vi "UI.vi"(8 "error in (no error)":errorcluster, 11 "Node Ptr":T1 format="%.0x") -> (0 "error out":errorcluster)   [LabVIEW 2020, in "Modules.lvlib" / "9210.lvclass"]
uses:
  9210.lvclass
  <vilib>/NI VeriStand/Custom Device API/Custom Device Item Ref.ctl
  RSI Module/SubPanel Command.ctl
  C:/Users/nitest/Desktop/Git 2020/niveristand-scan-engine-module-libraries/Source/RSI Module/RSI Module.lvclass
  9210.lvclass/9210.ctl
  RSI Module/RSI Module.lvclass
  <vilib>/NI VeriStand/Custom Device API/Custom Device API.lvlib
panel:
  in  "Units":u8(ring) caption="Measurement Units" items=["Raw Volts", "Degrees Kelvin", "Degrees Celsius", "Degrees Fahrenheit", "Degrees Rankine"]
  in  "Type":u8(ring) caption="Thermocouple Type" items=["J", "K", "T", "E", "R", "S", "N", "B"]
  in  "Channels":i32[](listbox)=[0]
  in  "SubPanel Event":refnum<user-event>
  in  "Header":cluster{"Section Name":string}={"Section Name"="NI 9210 Settings"}
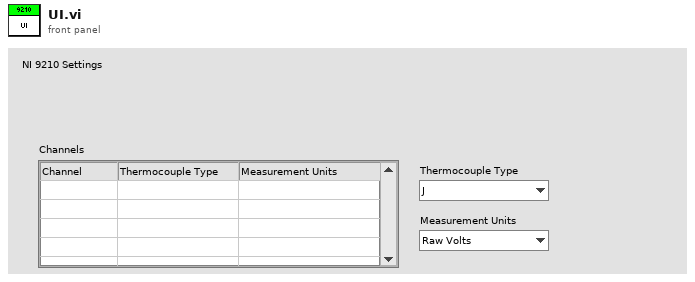
[diagram p1: front panel]
types:
  T1 = typedef "Custom Device API.lvlib/Custom Device Item Ref.ctl" = u64
  T2 = typedef "Modules.lvlib/RSI Module.lvclass/Module Models.ctl" = enum16{"Empty", "NI 9201", "NI 9203", "NI 9205", "NI 9206", "NI 9207", "NI 9208", "NI 9209", "NI 9210", "NI 9211", "NI 9212", "NI 9213", "NI 9214", "NI 9215", "NI 9216", "NI 9217", "NI 9219", "NI 9220", "NI 9221", "NI 9222", "NI 9223", "NI 9224", "NI 9225", "NI 9226", "NI 9227", "NI 9228", "NI 9229", "NI 9233", "NI 9234", "NI 9235", "NI 9236", "NI 9237", "NI 9239", "NI 9242", "NI 9244", "NI 9253", "NI 9263", "NI 9264", "NI 9265", "NI 9266", "NI 9269", "NI 9344", "NI 9350", "NI 9375", "NI 9401", "NI 9402", "NI 9403", "NI 9411", "NI 9421", "NI 9422", "NI 9423", "NI 9425", "NI 9426", "NI 9435", "NI 9436", "NI 9437", "NI 9472", "NI 9474", "NI 9475", "NI 9476", "NI 9477", "NI 9478", "NI 9481", "NI 9482", "NI 9485"}
  T3 = typedef "Modules.lvlib/RSI Module.lvclass/SubPanel Command.ctl" = enum16{"Stop"}
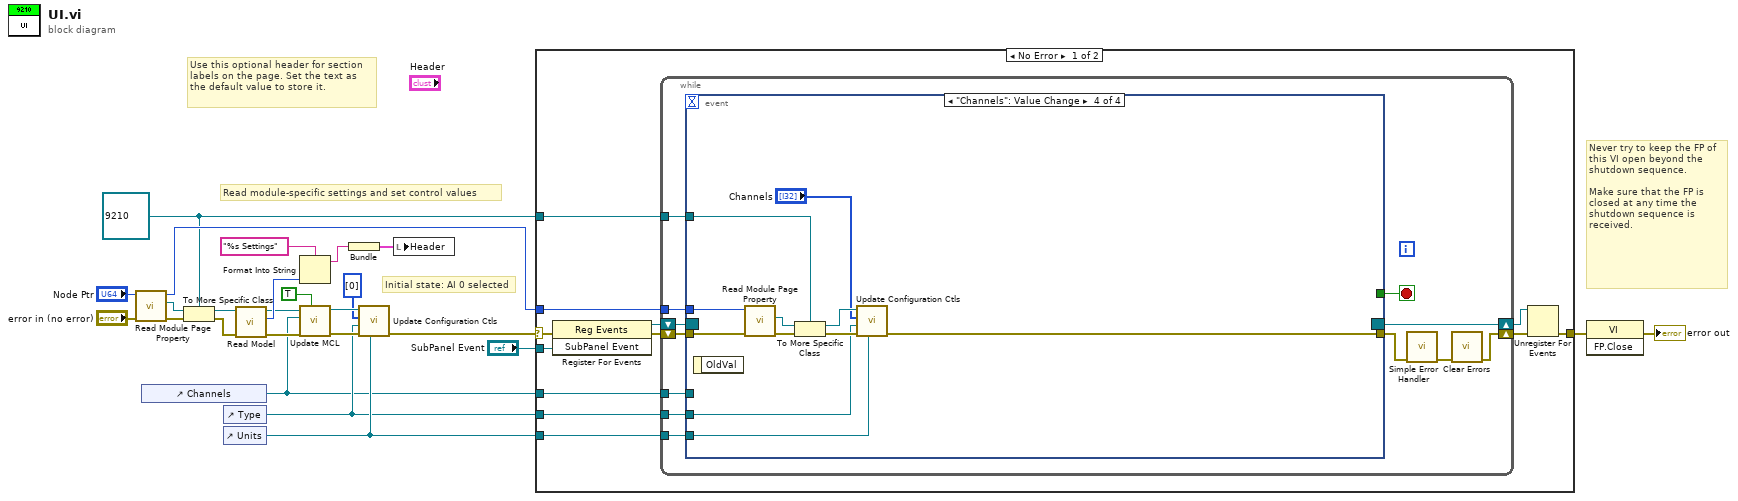
[diagram p0: block diagram]
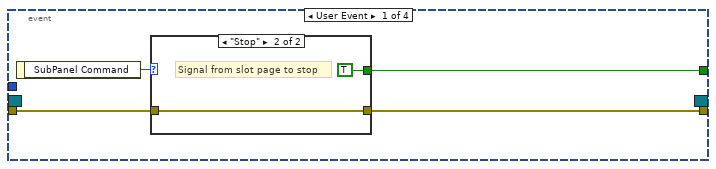
[diagram p2: hidden frame]
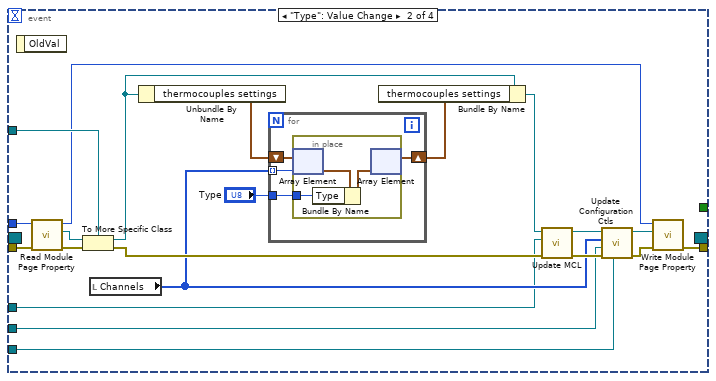
[diagram p4: hidden frame]
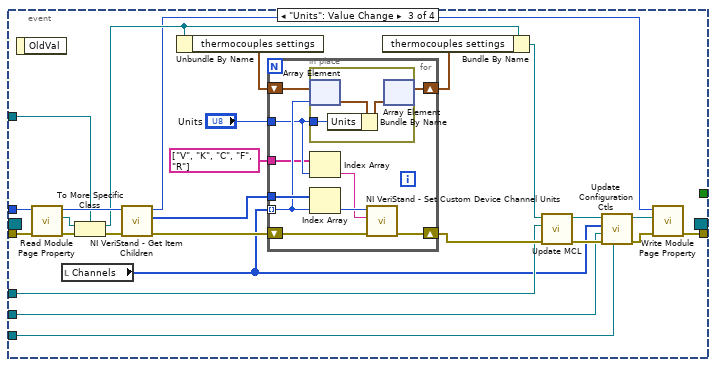
[diagram p5: hidden frame]
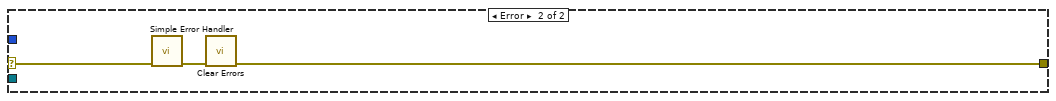
[diagram p6: hidden frame]
diagram:
  w2 = refnum<class "9210.lvclass"> refnum ("9205 in")
  # "Never try to keep the FP of this VI open beyond the shutdown sequence.\n\nMake sure that the FP is closed at any time the shutdown sequence is received."
  # "Initial state: AI 0 selected"
  # "Read module-specific settings and set control values"
  # "Use this optional header for section labels on the page. Set the text as the default value to store it."
  n1 = call "Read Module Page Property.vi"("error in (no error)"="error in (no error)", "Node Ptr In"="Node Ptr") -> ("error out"=w19:errorcluster, "RSI Module"=w18:refnum<class "RSI Module.lvclass">, "Node Ptr Out"=w22:T1)  [unwired: 7 in]
  n2 = control-ref of="Channels"() -> (w3:refnum<vi>)
  n3 = To More Specific Class(target class=w2, reference=w18, error in=w19) -> (specific class reference=w7:refnum<class "9210.lvclass">, error out=w8:errorcluster)
  n4 = control-ref of="Type"() -> (w4:refnum<vi>)
  n5 = control-ref of="Units"() -> (w5:refnum<vi>)
  n6 = call "Read Model.vi"("error in (no error)"=w8, "RSI Module in"=w7) -> ("error out"=w13:errorcluster, "Model"=w16:T2, "RSI Module out"=w12:refnum<class "9210.lvclass">)  [unwired: 7 in]
  n7 = Format Into String(format string="%s Settings", w16) -> (resulting string=w14:string)  [unwired: 2 in, 1 out]
  n8 = call "Update MCL.vi"("initialize MCL value"=TRUE, "error in"=w13, "MCL refnum"=w3, "9210 in"=w12) -> ("error out"=w11:errorcluster, "9210 out"=w10:refnum<class "9210.lvclass">)  [unwired: 6 in]
  n9 = Bundle(w14) -> (w17:cluster{string})  [unwired: 1 in]
  n10 = call "Update Configuration Ctls.vi"("Units"=w5, "error in"=w11, "Type"=w4, "selected channels"=i32[] [0] ("Selected Channels"), "9210 in"=w10) -> ("error out"=w6:errorcluster)  [unwired: 5 in, 1 out]
  n11 = local write "Header"(w17) -> ()
  n12 = case shown="No Error" w6 {
    selector: w6 -> [w31 w137]
    tunnel: [w35 w135] -> w25
    tunnel: w22 -> [w32 _]
    tunnel: "SubPanel Event" -> [w30 _]
    tunnel: w5 -> [w29 _]
    tunnel: w4 -> [w28 _]
    tunnel: w3 -> [w27 _]
    tunnel: w2 -> [w26 _]
    frame No Error {
      n13 = register-events(error in=w31, w30) -> (reference out=w33:refnum<event-registration>, error out=w34:errorcluster)  [unwired: 1 in]
      n14 = while {
        tunnel: w32 -> [w45]
        shift-right: [w42] -> w36
        shift-left: w34 -> [w48]
        shift-right: [w49] -> w37
        shift-left: w33 -> [w47]
        tunnel: w26 -> [w41]
        tunnel: w29 -> [w40]
        tunnel: w28 -> [w39]
        tunnel: w27 -> [w38]
        stop <- w46 stop-if-true
        n15 = event shown="[3] \"Channels\": Value Change" {
          selector: w47 -> [_ _ _ _]
          dyn-events: [_ _ _ _] -> w49
          timeout: _ -> [_ _ _ _]
          tunnel: w48 -> [w52 w74 w107 w132]
          tunnel: [w51 _ _ _] -> w46
          tunnel: [w50 w73 w106 w128] -> w44
          tunnel: w45 -> [_ w75 w108 w131]
          tunnel: w41 -> [_ w67 w94 w124]
          tunnel: w40 -> [_ w65 w90 w125]
          tunnel: w39 -> [_ w66 w89 w126]
          tunnel: w38 -> [_ w58 w88 _]
          event User Event {
            n16 = event-data() -> ("SubPanel Command"=w53:T3)  [unwired: 1 out]
            n17 = case shown="\"Stop\"" w53 {
              tunnel: w52 -> [w54 w55]
              tunnel: [w54 w55] -> w50
              tunnel: [_ TRUE] -> w51
              frame Default {
              }
              frame "Stop" {
                # "Signal from slot page to stop"
              }
            }
          }
          event "Type": Value Change {
            n18 = event-data() -> ()  [unwired: 2 out]
            n19 = call "Read Module Page Property.vi"("error in (no error)"=w74, "Node Ptr In"=w75) -> ("error out"=w76:errorcluster, "RSI Module"=w77:refnum<class "RSI Module.lvclass">, "Node Ptr Out"=w57:T1)  [unwired: 7 in]
            n20 = To More Specific Class(target class=w67, reference=w77, error in=w76) -> (specific class reference=w62:refnum<class "9210.lvclass">, error out=w72:errorcluster)
            n21 = local read "Channels"() -> (w59:i32[])
            n22 = Unbundle By Name(w62) -> ("thermocouples settings"=w64:cluster{"Units":u8, "Type":u8}[])
            n23 = for {
              tunnel: w59 -> [w80] mode=indexing
              shift-right: [w78] -> w63
              shift-left: w64 -> [w81]
              tunnel: "Type" -> [w79]
              n24 = in-place {
                in-place-border: w79 -> [w83]
                n25 = in-place-array #1(w81, w80) -> (w84:cluster{"Units":u8, "Type":u8})
                n26 = Bundle By Name(cluster=w84, "Type"=w83) -> (w82:cluster{"Units":u8, "Type":u8})
                n27 = in-place-array #1(w82) -> (w78:cluster{"Units":u8, "Type":u8}[])  [unwired: 1 out]
              }
            }
            n28 = Bundle By Name(cluster=w62, "thermocouples settings"=w63) -> (w61:refnum<class "9210.lvclass">)
            n29 = call "Update MCL.vi"("error in"=w72, "MCL refnum"=w58, "9210 in"=w61) -> ("error out"=w71:errorcluster, "9210 out"=w69:refnum<class "9210.lvclass">)  [unwired: 7 in]
            n30 = call "Update Configuration Ctls.vi"("Units"=w65, "error in"=w71, "Type"=w66, "selected channels"=w59, "9210 in"=w69) -> ("error out"=w70:errorcluster, "9210 out"=w68:refnum<class "9210.lvclass">)  [unwired: 5 in]
            n31 = call "Write Module Page Property.vi"("error in (no error)"=w70, "RSI Module"=w68, "Node Ptr In"=w57) -> ("error out"=w73:errorcluster)  [unwired: 6 in, 2 out]
          }
          event "Units": Value Change {
            n32 = event-data() -> ()  [unwired: 2 out]
            n33 = call "Read Module Page Property.vi"("error in (no error)"=w107, "Node Ptr In"=w108) -> ("error out"=w109:errorcluster, "RSI Module"=w110:refnum<class "RSI Module.lvclass">, "Node Ptr Out"=w99:T1)  [unwired: 7 in]
            n34 = local read "Channels"() -> (w87:i32[])
            n35 = To More Specific Class(target class=w94, reference=w110, error in=w109) -> (specific class reference=w86:refnum<class "9210.lvclass">, error out=w100:errorcluster)
            n36 = call <vilib>:"NI VeriStand - Get Item Children.vi"("error in (no error)"=w100, "Item Ref in"=w99) -> ("error out"=w97:errorcluster, "Child Refs"=w98:T1[], "Item Ref out"=w85:T1)  [unwired: 6 in, 1 out]
            n37 = Unbundle By Name(w86) -> ("thermocouples settings"=w93:cluster{"Units":u8, "Type":u8}[])
            n38 = for {
              tunnel: w87 -> [w114] mode=indexing
              shift-right: [w112] -> w92
              shift-left: w93 -> [w115]
              tunnel: "Units" -> [w113]
              shift-right: [w117] -> w96
              shift-left: w97 -> [w118]
              tunnel: w98 -> [w120]
              tunnel: string[] ["V", "K", "C", "F", "R"] -> [w111]
              n39 = in-place {
                in-place-border: w113 -> [w122]
                n40 = in-place-array #2(w115, w114) -> (w123:cluster{"Units":u8, "Type":u8})
                n41 = Bundle By Name(cluster=w123, "Units"=w122) -> (w121:cluster{"Units":u8, "Type":u8})
                n42 = in-place-array #2(w121) -> (w112:cluster{"Units":u8, "Type":u8}[])  [unwired: 1 out]
              }
              n43 = Index Array(array=w111, index=w113) -> (element=w116:string)
              n44 = Index Array(array=w120, index=w114) -> (element=w119:T1)
              n45 = call <vilib>:"NI VeriStand - Set Custom Device Channel Units.vi"("error in (no error)"=w118, "Units"=w116, "Channel Ref in"=w119) -> ("error out"=w117:errorcluster)  [unwired: 7 in, 1 out]
            }
            n46 = Bundle By Name(cluster=w86, "thermocouples settings"=w92) -> (w91:refnum<class "9210.lvclass">)
            n47 = call "Update MCL.vi"("error in"=w96, "MCL refnum"=w88, "9210 in"=w91) -> ("error out"=w105:errorcluster, "9210 out"=w103:refnum<class "9210.lvclass">)  [unwired: 7 in]
            n48 = call "Update Configuration Ctls.vi"("Units"=w90, "error in"=w105, "Type"=w89, "selected channels"=w87, "9210 in"=w103) -> ("error out"=w104:errorcluster, "9210 out"=w101:refnum<class "9210.lvclass">)  [unwired: 5 in]
            n49 = call "Write Module Page Property.vi"("error in (no error)"=w104, "RSI Module"=w101, "Node Ptr In"=w85) -> ("error out"=w106:errorcluster)  [unwired: 6 in, 2 out]
          }
          event "Channels": Value Change {
            n50 = event-data() -> ()  [unwired: 2 out]
            n51 = call "Read Module Page Property.vi"("error in (no error)"=w132, "Node Ptr In"=w131) -> ("error out"=w133:errorcluster, "RSI Module"=w134:refnum<class "RSI Module.lvclass">)  [unwired: 7 in, 1 out]
            n52 = To More Specific Class(target class=w124, reference=w134, error in=w133) -> (specific class reference=w129:refnum<class "9210.lvclass">, error out=w130:errorcluster)
            n53 = call "Update Configuration Ctls.vi"("Units"=w125, "error in"=w130, "Type"=w126, "selected channels"="Channels", "9210 in"=w129) -> ("error out"=w128:errorcluster)  [unwired: 5 in, 1 out]
          }
        }
        n54 = call <vilib>:"Simple Error Handler.vi"("error in (no error)"=w44) -> ("error out"=w43:errorcluster)  [unwired: 1 in, 7 out]
        n55 = call <vilib>:"Clear Errors.vi"("error in (no error)"=w43) -> ("error out"=w42:errorcluster)  [unwired: 1 in, 5 out]
      }
      n56 = Unregister For Events(event registration refnum=w37, error in=w36) -> (error out=w35:errorcluster)
    }
    frame Error {
      n57 = call <vilib>:"Simple Error Handler.vi"("error in (no error)"=w137) -> ("error out"=w136:errorcluster)  [unwired: 1 in, 7 out]
      n58 = call <vilib>:"Clear Errors.vi"("error in (no error)"=w136) -> ("error out"=w135:errorcluster)  [unwired: 1 in, 5 out]
    }
  }
  n59 = invoke class="VI" method="FP.Close"(error in=w25) -> (error out=→"error out":errorcluster)  [unwired: 2 in, 2 out]
